vi "Close.vi"(8 "error in":errorcluster, 11 "ToastBuilder in":refnum<class "ToastBuilder.lvclass">) -> (0 "error out":errorcluster)   [LabVIEW 2026, in "ToastNotification.lvlib" / "ToastBuilder.lvclass"]
doc: "ToastSource cleanup override for ToastBuilder. Executes even on incoming error: attempt to close the native builder reference and merge the incoming error before cleanup failures. Empty and already closed handles are ignored by the release helper. Closing one alias invalidates all copies of the handle. Does not unregister ToastService callbacks or collect the .NET heap."
uses:
  ToastBuilder.lvclass
  ToastBuilder.lvclass/ToastBuilder.ctl
  Read Builder Reference.vi
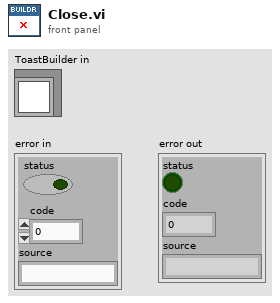
[diagram p1: front panel]
types:
  T1 = typedef "ToastNotification.lvlib/ToastBuilder.lvclass/Builder Reference.ctl" = refnum<k24>
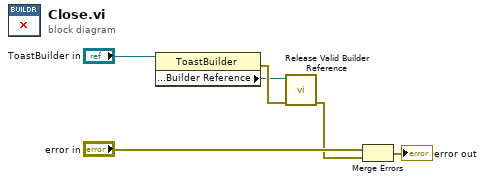
[diagram p0: block diagram]
diagram:
  n1 = property class="ToastBuilder"(reference="ToastBuilder in") -> (error out=w3:errorcluster, "Public:Properties:Builder Reference"=w2:T1)  [unwired: 1 in, 1 out]
  n2 = call "Release Valid Builder Reference.vi"("error in (no error)"=w3, "reference"=w2) -> ("error out"=w1:errorcluster)  [unwired: 9 in]
  n3 = Merge Errors("error in", w1) -> (→"error out":errorcluster)
